vi "Add Error Core.vi"(8 "error in (no error)":errorcluster, 10 "String to Append":string, 11 "Error":T1) -> (0 "error out":errorcluster)   [LabVIEW 2021, in "CAN_Writer_NIXNET_Common.lvlib"]
uses:
  CAN_Writer_NIXNET_Common.lvlib
  <vilib>/CIF Foundation/CIF Utilities/Errors/Errors_CIF_U.lvlib
  Typedef/Errors.ctl
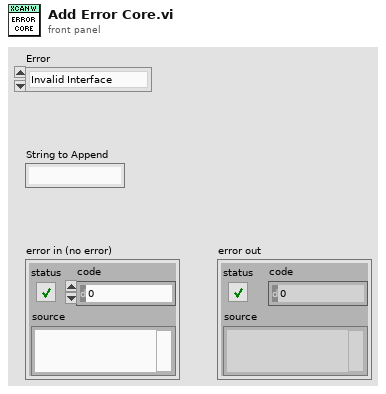
[diagram p1: front panel]
types:
  T1 = typedef "CAN_Writer_NIXNET_Common.lvlib/Errors.ctl" = enum16{"Invalid Interface"}
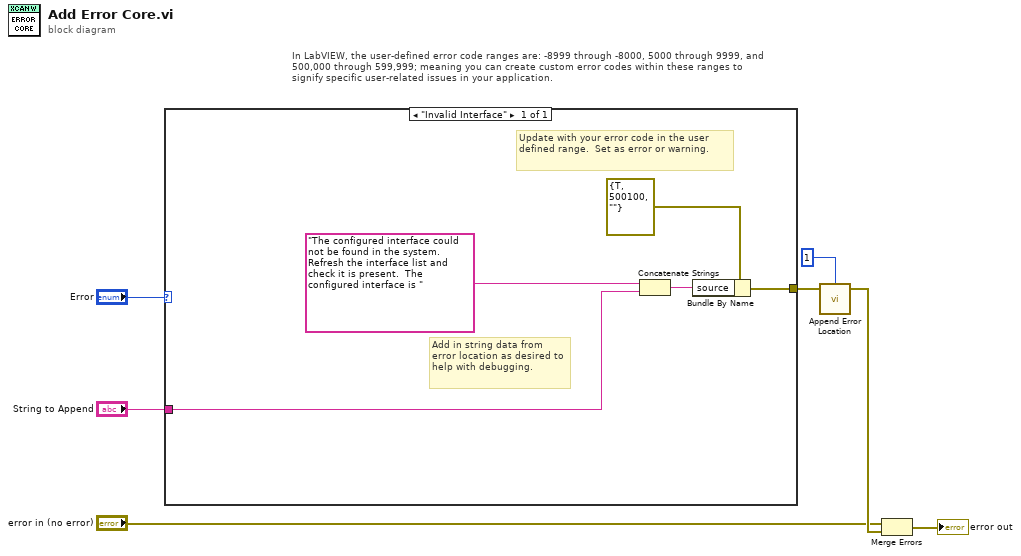
[diagram p0: block diagram]
diagram:
  # "In LabVIEW, the user-defined error code ranges are: -8999 through -8000, 5000 through 9999, and 500,000 through 599,999; meaning you can create custom error codes within these ranges to signify specific user-related issues in your application."
  n1 = case shown="\"Invalid Interface\"" "Error" {
    tunnel: "String to Append" -> [w9]
    tunnel: [w11] -> w6
    frame "Invalid Interface" {
      # "Add in string data from error location as desired to help with debugging."
      # "Update with your error code in the user defined range.  Set as error or warning."
      n2 = Concatenate Strings("The configured interface could not be found in the system. Refresh the interface list and check it is present.  The configured interface is " ("source"), w9) -> (w8:string)
      n3 = Bundle By Name(cluster=errorcluster {"status"=TRUE, "code"=500100, "source"=""} ("Invalid ID"), "source"=w8) -> (w11:errorcluster)
    }
  }
  n4 = call <vilib>:"Append Error Location.vi"("error in (no error)"=w6, "Chain Depth"=1) -> ("error out"=w7:errorcluster)  [unwired: 3 in]
  n5 = Merge Errors("error in (no error)", w7) -> (→"error out":errorcluster)
